vi "Move Turn Table.vi"(8 "error in (no error)":errorcluster, 11 "ETS_EM2090 in":refnum<class "ETS_EM2090.lvclass">) -> (0 "error out":errorcluster, 3 "ETS_EM2090 out":refnum<class "ETS_EM2090.lvclass">)   [LabVIEW 2023, in "Turn Table and Mast.lvlib" / "ETS_EM2090.lvclass"]
uses:
  ETS_EM2090.lvclass
  ETS_EM2090.lvclass/ETS_EM2090.ctl
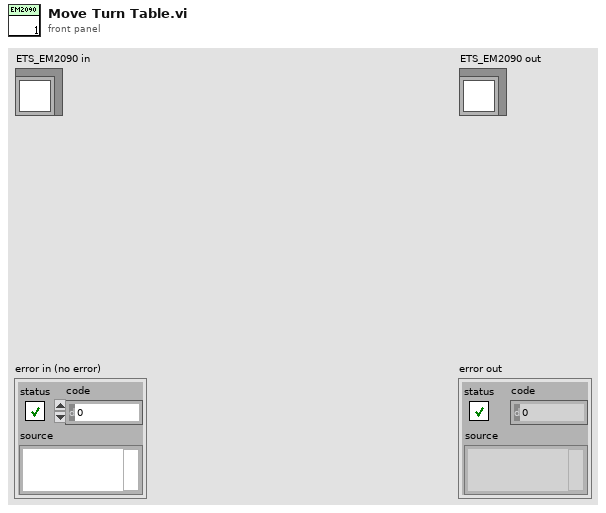
[diagram p1: front panel]
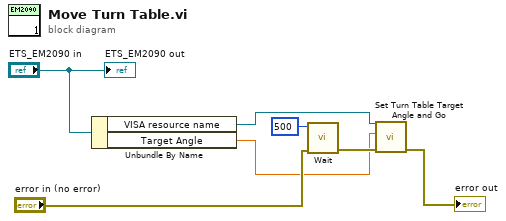
[diagram p0: block diagram]
diagram:
  n1 = Unbundle By Name("ETS_EM2090 in") -> ("VISA resource name"=w2:refnum<visa-resource-name>, "Target Angle"=w1:dbl)
  n2 = call "Wait.vi"("에러 상수 입력"="error in (no error)", "대기 시간 (ms)"=u32 500) -> ("에러 상수 출력"=w4:errorcluster)  [unwired: 9 in]
  n3 = call "Set Turn Table Target Angle and Go.vi"("error in (no error)"=w4, "Target Angle"=w1, "VISA Refnum in"=w2) -> ("error out"=→"error out":errorcluster)  [unwired: 7 in, 1 out]
  "ETS_EM2090 out" <- "ETS_EM2090 in"
